vi "Configure.vi"(8 "error in (no error)":errorcluster, 10 "vi path":path=path "Default settings.vi", 11 "HamamatsuFluor in":refnum<class "HamamatsuFluor.lvclass">) -> (0 "error out":errorcluster, 3 "HamamatsuFluor out":refnum<class "HamamatsuFluor.lvclass">)   [LabVIEW 2020, in "DAQ Timed SPIM.lvlib" / "HamamatsuFluor_v2.lvlib" / "HamamatsuFluor.lvclass"]
uses:
  HamamatsuFluor.lvclass
  HamamatsuFluor.lvclass/HamamatsuFluor.ctl
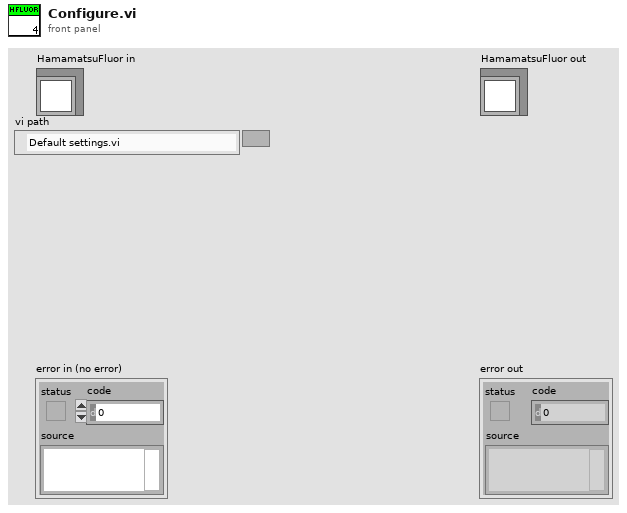
[diagram p1: front panel]
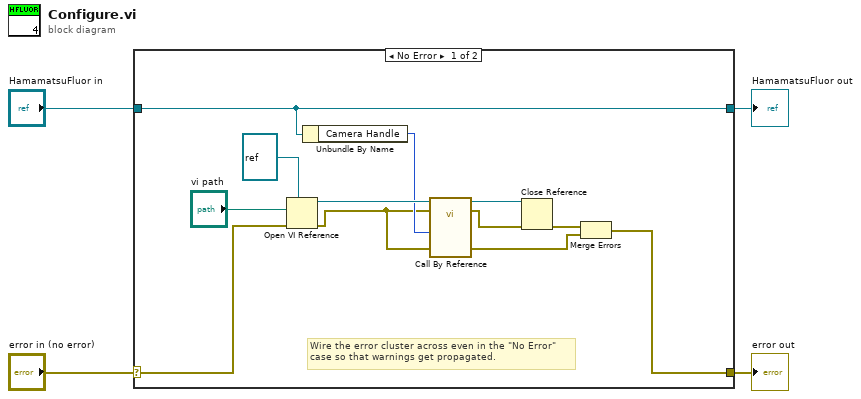
[diagram p0: block diagram]
diagram:
  n1 = case shown="No Error" "error in (no error)" {
    selector: "error in (no error)" -> [w11 w18]
    tunnel: [w5 w18] -> w3
    tunnel: [w13 w17] -> w1
    tunnel: "HamamatsuFluor in" -> [w13 w17]
    frame No Error {
      # "Wire the error cluster across even in the \"No Error\"\ncase so that warnings get propagated."
      n2 = Open VI Reference(type specifier VI Refnum (for type only)=refnum<vi> refnum, vi path="vi path", error in (no error)=w11) -> (vi reference=w14:refnum<vi>, error out=w8:errorcluster)  [unwired: 3 in]
      n3 = Unbundle By Name(w13) -> ("Camera Handle"=w12:u32)
      n4 = call-by-ref "?"(reference=w14, error in=w8, 8:"error in (no error)"=w8, "Camera handle"=w12) -> (reference out=w10:refnum<vi>, error out=w9:errorcluster, 0:"error out"=w6:errorcluster)  [unwired: 9 in]
      n5 = Close Reference(reference=w10, error in (no error)=w9) -> (error out=w7:errorcluster)
      n6 = Merge Errors(w7, w6) -> (w5:errorcluster)
    }
    frame Error {
    }
  }
  "error out" <- w3
  "HamamatsuFluor out" <- w1
